vi "Init ensemble var glob.vi"() -> (0 "error out":errorcluster caption="sortie d'erreur")   [LabVIEW 2022 SP3]
uses:
  Pressions/Gestion grappe/TypeDef_Seuil Jauge Pression_CN.ctl
  Variables globales/Variable glob generale.vi
  Variables globales/Variable glob mails.vi
  Variables globales/Variable glob Leybold.vi
  Variables globales/Variable glob Edwards.vi
  Variables globales/Variable glob alertes pressions.vi
  Variables globales/Variable glob Th.vi
  Variables globales/Variable glob Pt.vi
  Variables globales/Variable glob alertes min-max temperatures.vi
  Variables globales/Variable glob alertes ecart temperatures.vi
  Variables globales/Variables glob EUROTHERM.vi
  Variables globales/Variable glob Keller.vi
  Variables globales/Variable glob alertes Keller.vi
  Variables globales/Variable glob alertes Compteurs.vi
  Variables globales/Variable globale compteurs.vi
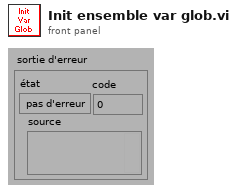
[diagram p1: front panel]
types:
  T1 = typedef "TypeDef_Seuil Jauge Pression_CN.ctl" = cluster{"Descente en Pression":cluster{"Min Mesure Piezo":dbl, "Min Mesure Pirani":dbl}, "Montée en Pression":cluster{"Max Mesure Pirani":dbl, "Max Mesure Penning":dbl}}
  T2 = cluster{"Alerte":bool, "valeur ":dbl, "Défaut":bool, "Indices controler":i16[], "N°":u16}[]
  T3 = cluster{"Nom tache Th":refnum<k21>, "Noms des Th":string[], "Nb Th":i16, "Sélection Th":bool[], "Nom Th sélectionnées":string[]}[]
  T4 = cluster{"Nom tache Pt":refnum<k21>, "Noms des Pt":string[], "Nb Pt":i16, "Sélection Pt":bool[], "Nom Pt sélectionnées":string[]}[]
  T5 = cluster{"Alerte temp min/max":bool, "température max":dbl, "température min":dbl, "Défaut min/max temp":bool, "Indices à controler":i16[], "N°":u16}[]
  T6 = cluster{"Indices a controler":i16[], "Defaut":bool, "ecart temp":dbl, "Alerte":bool, ">?":bool, "N°":u16}[]
  T7 = cluster{"Alerte Keller":bool, "valeur alerte Keller":dbl, "Défaut Keller":bool, "Indices Keller à controler":i16[], "N°":u16}[]
  T8 = cluster{"Alerte":bool, "valeur alerte":dbl, "Défaut":bool, "Indices à controler":i16[], "N°":u16}[]
  T9 = cluster{"Nom tache compteurs":refnum<k21>, "Noms des compteurs":string[], "Sélection":bool[], "Init compteurs":dbl[], "Noms compteurs sélectionnés":string[]}
  T10 = typedef "Semaphore RefNum" = refnum<k1>
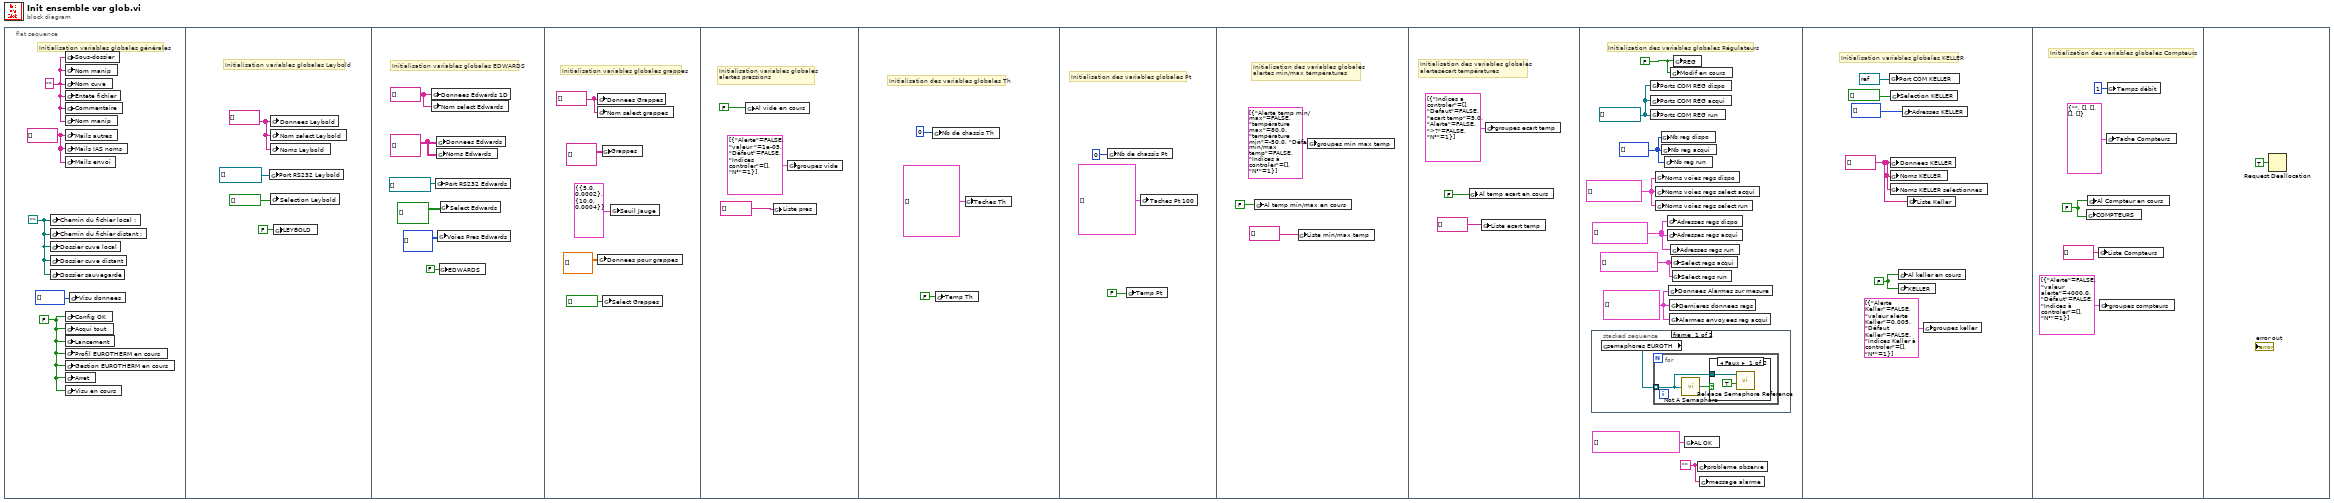
[diagram p0: block diagram]
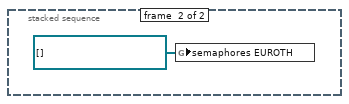
[diagram p3: hidden frame]
diagram:
  n1 = flat-sequence {
    frame #0 {
      w1 = string[] [] ("Mails autres")
      w2 = FALSE ("Acqui tout")
      w3 = "" ("Nom cuve")
      w5 = path ""
      # "Initialisation variables globales générales"
      n2 = global write "Variable glob generale.vi" "Chemin du fichier local :"(w5) -> ()
      n3 = global write "Variable glob generale.vi" "Chemin du fichier distant :"(w5) -> ()
      n4 = global write "Variable glob generale.vi" "Dossier cuve local"(w5) -> ()
      n5 = global write "Variable glob generale.vi" "Dossier cuve distant"(w5) -> ()
      n6 = global write "Variable glob generale.vi" "Dossier sauvegarde"(w5) -> ()
      n7 = global write "Variable glob generale.vi" "Sous-dossier"(w3) -> ()
      n8 = global write "Variable glob generale.vi" "Nom manip"(w3) -> ()
      n9 = global write "Variable glob generale.vi" "Nom cuve"(w3) -> ()
      n10 = global write "Variable glob generale.vi" "Entete fichier"(w3) -> ()
      n11 = global write "Variable glob generale.vi" "Commentaire"(w3) -> ()
      n12 = global write "Variable glob generale.vi" "Nom manip"(w3) -> ()
      n13 = global write "Variable glob mails.vi" "Mails autres"(w1) -> ()
      n14 = global write "Variable glob mails.vi" "Mails IAS noms"(w1) -> ()
      n15 = global write "Variable glob mails.vi" "Mails envoi"(w1) -> ()
      n16 = global write "Variable glob generale.vi" "Config OK"(w2) -> ()
      n17 = global write "Variable glob generale.vi" "Acqui tout"(w2) -> ()
      n18 = global write "Variable glob generale.vi" "Lancement"(w2) -> ()
      n19 = global write "Variable glob generale.vi" "Profil EUROTHERM en cours"(w2) -> ()
      n20 = global write "Variable glob generale.vi" "Gestion EUROTHERM en cours"(w2) -> ()
      n21 = global write "Variable glob generale.vi" "Arret"(w2) -> ()
      n22 = global write "Variable glob generale.vi" "Visu en cours"(w2) -> ()
      n23 = global write "Variable glob generale.vi" "Visu donnees"(i32[] [] ("Visu données")) -> ()
    }
    frame #1 {
      w6 = string[] [] ("Noms jauges")
      # "Initialisation variables globales Leybold"
      n24 = global write "Variable glob Leybold.vi" "Port RS232 Leybold"(refnum<visa-resource-name>[] [] ("Port RS232 Edwards")) -> ()
      n25 = global write "Variable glob Leybold.vi" "Donnees Leybold"(w6) -> ()
      n26 = global write "Variable glob Leybold.vi" "Nom select Leybold"(w6) -> ()
      n27 = global write "Variable glob Leybold.vi" "Noms Leybold"(w6) -> ()
      n28 = global write "Variable glob Leybold.vi" "Selection Leybold"(bool[] [] ("Sélection jauges")) -> ()
      n29 = global write "Variable glob Leybold.vi" "LEYBOLD"(FALSE ("Alerte pression")) -> ()
    }
    frame #2 {
      w10 = string[] [] ("Nom sélect Edwards")
      w11 = string[][] [] ("Noms jauges")
      # "Initialisation variables globales EDWARDS"
      n30 = global write "Variable glob Edwards.vi" "Donnees Edwards 1D"(w10) -> ()
      n31 = global write "Variable glob Edwards.vi" "Nom select Edwards"(w10) -> ()
      n32 = global write "Variable glob Edwards.vi" "Port RS232 Edwards"(refnum<visa-resource-name>[] [] ("Port RS232 Edwards")) -> ()
      n33 = global write "Variable glob Edwards.vi" "Donnees Edwards"(w11) -> ()
      n34 = global write "Variable glob Edwards.vi" "Noms Edwards"(w11) -> ()
      n35 = global write "Variable glob Edwards.vi" "Voies Pres Edwards"(i8[][] [] ("Voies Pressions")) -> ()
      n36 = global write "Variable glob Edwards.vi" "EDWARDS"(FALSE ("EDWARDS")) -> ()
      n37 = global write "Variable glob Edwards.vi" "Select Edwards"(bool[][] [] ("Sélection jauges")) -> ()
    }
    frame #3 {
      w20 = string[] [] ("Nom sélect Edwards")
      # "Initialisation variables globales grappes"
      n38 = global write "Variable glob Edwards.vi" "Donnees Grappes"(w20) -> ()
      n39 = global write "Variable glob Edwards.vi" "Nom select grappes"(w20) -> ()
      n40 = global write "Variable glob Edwards.vi" "Donnees pour grappes"(dbl[][] [] ("Données pour grappes")) -> ()
      n41 = global write "Variable glob Edwards.vi" "Grappes"(string[][] [] ("Grappes")) -> ()
      n42 = global write "Variable glob Edwards.vi" "Select Grappes"(bool[] [] ("Sélect Grappes")) -> ()
      n43 = global write "Variable glob Edwards.vi" "Seuil Jauge"(T1 {"Descente en Pression"={"Min Mesure Piezo"=5.0, "Min Mesure Pirani"=0.0002}, "Montée en Pression"={"Max Mesure Pirani"=10.0, "Max Mesure Penning"=0.0004}} ("Seuil Jauge")) -> ()
    }
    frame #4 {
      # "Initialisation variables globales \nalertes pressions"
      n44 = global write "Variable glob alertes pressions.vi" "Al vide en cours"(FALSE ("Alerte pression")) -> ()
      n45 = global write "Variable glob alertes pressions.vi" "Liste pres"(string[] [] ("Mail alerte pressions")) -> ()
      n46 = global write "Variable glob alertes pressions.vi" "groupes vide"(T2 [{"Alerte"=FALSE, "valeur "=1e-05, "Défaut"=FALSE, "Indices controler"=[], "N°"=1}] ("groupes vide")) -> ()
    }
    frame #5 {
      # "Initialisation des variables globales Th"
      n47 = global write "Variable glob Th.vi" "Nb de chassis Th"(u8 0 ("Nombre de chassis SCXI")) -> ()
      n48 = global write "Variable glob Th.vi" "Temp Th"(FALSE ("SCXI")) -> ()
      n49 = global write "Variable glob Th.vi" "Taches Th"(T3 [] ("Taches Th")) -> ()
    }
    frame #6 {
      # "Initialisation des variables globales Pt"
      n50 = global write "Variable glob Pt.vi" "Nb de chassis Pt"(u8 0 ("Nombre de modules Pt")) -> ()
      n51 = global write "Variable glob Pt.vi" "Temp Pt"(FALSE) -> ()
      n52 = global write "Variable glob Pt.vi" "Taches Pt 100"(T4 [] ("Taches Pt 100")) -> ()
    }
    frame #7 {
      # "Initialisation des variables globales \nalertes min/max températures"
      n53 = global write "Variable glob alertes min-max temperatures.vi" "Al temp min/max en cours"(FALSE ("Alerte temp min/max")) -> ()
      n54 = global write "Variable glob alertes min-max temperatures.vi" "Liste min/max temp"(string[] [] ("Liste min/max temp")) -> ()
      n55 = global write "Variable glob alertes min-max temperatures.vi" "groupes min max temp"(T5 [{"Alerte temp min/max"=FALSE, "température max"=80.0, "température min"=-50.0, "Défaut min/max temp"=FALSE, "Indices à controler"=[], "N°"=1}] ("groupes min max temp")) -> ()
    }
    frame #8 {
      # "Initialisation des variables globales \nalertesécart températures"
      n56 = global write "Variable glob alertes ecart temperatures.vi" "Al temp ecart en cours"(FALSE ("Alerte temp écart")) -> ()
      n57 = global write "Variable glob alertes ecart temperatures.vi" "Liste ecart temp"(string[] [] ("Liste ecart temp")) -> ()
      n58 = global write "Variable glob alertes ecart temperatures.vi" "groupes ecart temp"(T6 [{"Indices a controler"=[], "Defaut"=FALSE, "ecart temp"=5.0, "Alerte"=FALSE, ">?"=FALSE, "N°"=1}] ("groupes ecart temp")) -> ()
    }
    frame #9 {
      w38 = ""
      w40 = u8[] [] ("Nb reg acqui")
      w37 = cluster{"Dernières données 1COM":string[][]}[] [] ("Dernières données regs")
      w44 = cluster{"Sélect acqui 1COM reg":bool[]}[] [] ("Sélect regs acqui")
      w42 = cluster{"Adresses 1COM reg":u16[]}[] [] ("Adresses regs dispo")
      w43 = cluster{"Noms voies dispo 1COM":string[]}[] [] ("Noms voies regs dispo")
      w41 = refnum<visa-resource-name>[] [] ("Ports COM REG")
      w36 = FALSE ("REG")
      # "Initialisation des variables globales Régulateurs"
      n59 = stacked-sequence {
        frame #0 {
          n60 = global read "Variables glob EUROTHERM.vi" "semaphores EUROTH"() -> (w45:T10[])
          n61 = for {
            tunnel: w45 -> [w46] mode=indexing
            n62 = call <vilib>:"Not A Semaphore.vi"("semaphore"=w46) -> ("not a semaphore"=w47:bool)
            n63 = case shown="Faux" w47 {
              tunnel: w46 -> [w48 _]
              frame False {
                n64 = call <vilib>:"Release Semaphore Reference.vi"("force destroy? (F)"=TRUE, "semaphore"=w48) -> ()  [unwired: 8 in, 2 out]
              }
              frame True {
              }
            }
          }
        }
        frame #1 {
          w50 = T10[] [] items=["semaphore"] ("semaphores EUROTH")
          n65 = global write "Variables glob EUROTHERM.vi" "semaphores EUROTH"(w50) -> ()
        }
      }
      n66 = global write "Variables glob EUROTHERM.vi" "Ports COM REG dispo"(w41) -> ()
      n67 = global write "Variables glob EUROTHERM.vi" "Ports COM REG acqui"(w41) -> ()
      n68 = global write "Variables glob EUROTHERM.vi" "Ports COM REG run"(w41) -> ()
      n69 = global write "Variables glob EUROTHERM.vi" "Noms voies regs dispo"(w43) -> ()
      n70 = global write "Variables glob EUROTHERM.vi" "Noms voies regs select acqui"(w43) -> ()
      n71 = global write "Variables glob EUROTHERM.vi" "Noms voies regs select run"(w43) -> ()
      n72 = global write "Variables glob EUROTHERM.vi" "Nb reg dispo"(w40) -> ()
      n73 = global write "Variables glob EUROTHERM.vi" "Nb reg acqui"(w40) -> ()
      n74 = global write "Variables glob EUROTHERM.vi" "Nb reg run"(w40) -> ()
      n75 = global write "Variables glob EUROTHERM.vi" "Adresses regs dispo"(w42) -> ()
      n76 = global write "Variables glob EUROTHERM.vi" "Adresses regs acqui"(w42) -> ()
      n77 = global write "Variables glob EUROTHERM.vi" "Donnees Alarmes sur mesure"(w37) -> ()
      n78 = global write "Variables glob EUROTHERM.vi" "Dernieres donnees regs"(w37) -> ()
      n79 = global write "Variables glob EUROTHERM.vi" "Alarmes envoyees reg acqui"(w37) -> ()
      n80 = global write "Variables glob EUROTHERM.vi" "Modif en cours"(w36) -> ()
      n81 = global write "Variables glob EUROTHERM.vi" "Adresses regs run"(w42) -> ()
      n82 = global write "Variables glob EUROTHERM.vi" "Select regs acqui"(w44) -> ()
      n83 = global write "Variables glob EUROTHERM.vi" "Select regs run"(w44) -> ()
      n84 = global write "Variables glob EUROTHERM.vi" "REG"(w36) -> ()
      n85 = global write "Variables glob EUROTHERM.vi" "AL OK"(cluster{"AL OK 1 COM":u16[]}[] [] ("AL OK")) -> ()
      n86 = global write "Variables glob EUROTHERM.vi" "probleme observe"(w38) -> ()
      n87 = global write "Variables glob EUROTHERM.vi" "message alarme"(w38) -> ()
    }
    frame #10 {
      w56 = FALSE ("Alerte Keller")
      w52 = string[] [] ("Noms KELLER")
      # "Initialisation variables globales KELLER"
      n88 = global write "Variable glob Keller.vi" "Port COM KELLER"(refnum<visa-resource-name> refnum ("Port RS232 Edwards")) -> ()
      n89 = global write "Variable glob Keller.vi" "Donnees KELLER"(w52) -> ()
      n90 = global write "Variable glob Keller.vi" "Noms KELLER"(w52) -> ()
      n91 = global write "Variable glob Keller.vi" "Noms KELLER selectionnes"(w52) -> ()
      n92 = global write "Variable glob Keller.vi" "Selection KELLER"(bool[] [] ("Sélection KELLER")) -> ()
      n93 = global write "Variable glob alertes Keller.vi" "Al keller en cours"(w56) -> ()
      n94 = global write "Variable glob Keller.vi" "KELLER"(w56) -> ()
      n95 = global write "Variable glob Keller.vi" "Adresses KELLER"(i32[] [] ("Adresses KELLER")) -> ()
      n96 = global write "Variable glob alertes Keller.vi" "Liste Keller"(w52) -> ()
      n97 = global write "Variable glob alertes Keller.vi" "groupes keller"(T7 [{"Alerte Keller"=FALSE, "valeur alerte Keller"=0.005, "Défaut Keller"=FALSE, "Indices Keller à controler"=[], "N°"=1}] ("groupes keller")) -> ()
    }
    frame #11 {
      w59 = FALSE ("COMPTEURS")
      # "Initialisation des variables globales Compteurs"
      n98 = global write "Variable globale compteurs.vi" "COMPTEURS"(w59) -> ()
      n99 = global write "Variable glob alertes Compteurs.vi" "Al Compteur en cours"(w59) -> ()
      n100 = global write "Variable glob alertes Compteurs.vi" "Liste Compteurs"(string[] [] ("Liste Compteurs")) -> ()
      n101 = global write "Variable glob alertes Compteurs.vi" "groupes compteurs"(T8 [{"Alerte"=FALSE, "valeur alerte"=4000.0, "Défaut"=FALSE, "Indices à controler"=[], "N°"=1}] ("groupes compteurs")) -> ()
      n102 = global write "Variable globale compteurs.vi" "Tache Compteurs"(T9 {"Nom tache compteurs"="", "Noms des compteurs"=[], "Sélection"=[], "Init compteurs"=[], "Noms compteurs sélectionnés"=[]} ("Tache Compteurs")) -> ()
      n103 = global write "Variable globale compteurs.vi" "Temps débit"(u16 1 ("Temps débit")) -> ()
    }
    frame #12 {
      n104 = Request Deallocation(TRUE ("flag")) -> ()
    }
  }
